vi "Anal tdms each save.vi"(5 "B Table":string[][](table), 6 "R Table":string[][](table), 7 "S Table":string[][](table), 8 "error in":errorcluster, 10 "Table Tag C":T1, 11 "TDMSファイル in":refnum<k34>) -> (0 "error out":errorcluster, 3 "TDMSファイル out":refnum<k34>)   [LabVIEW 2018]
panel:
  out "B Table Tag":string[](array[string])=["S # [n]", "S Peak Position [s]", "Signal [pA]", "Region BL [pA]", "Region STD [pA]", "Threshold [pA]", "Signal S [s]", "Signal E (s)", "S TL [ms]", "S DL [s]", "Bias [V]", "RT BL [pA]", "Chip ID [a]", "Ex ID [a]", "Distance [nm]", "EP1 [mV]", "EP2  [mV]", "Read Region Point [n", "STD [select]", "RT BL [select]", "RT STD [select]", "Moving Point [n]", "U threshold [n]", "D thereshold [n]", "STD smooth [n]", "Signal Region Point [n]", "H1 [n]", "H2 [n]"]
  out "R Table Tag":string[](array[string])=["S # [n]", "S Peak Position [s]", "Signal [pA]", "Region BL [pA]", "Region STD [pA]", "Threshold [pA]", "Signal S [s]", "Signal E (s)", "S TL [ms]", "S DL [s]", "Bias [V]", "RT BL [pA]", "Chip ID [a]", "Ex ID [a]", "Distance [nm]", "EP1 [mV]", "EP2  [mV]", "Read Region Point [n", "STD [select]", "RT BL [select]", "RT STD [select]", "Moving Point [n]", "U threshold [n]", "D thereshold [n]", "STD smooth [n]", "Signal Region Point [n]", "H1 [n]", "H2 [n]"]
  out "S Table Tag":string[](array[string])=["S # [n]", "S Peak Position [s]", "Signal [pA]", "Region BL [pA]", "Region STD [pA]", "Threshold [pA]", "Signal S [s]", "Signal E (s)", "S TL [ms]", "S DL [s]", "Bias [V]", "RT BL [pA]", "Chip ID [a]", "Ex ID [a]", "Distance [nm]", "EP1 [mV]", "EP2  [mV]", "Read Region Point [n", "STD [select]", "RT BL [select]", "RT STD [select]", "Moving Point [n]", "U threshold [n]", "D thereshold [n]", "STD smooth [n]", "Signal Region Point [n]", "H1 [n]", "H2 [n]"]
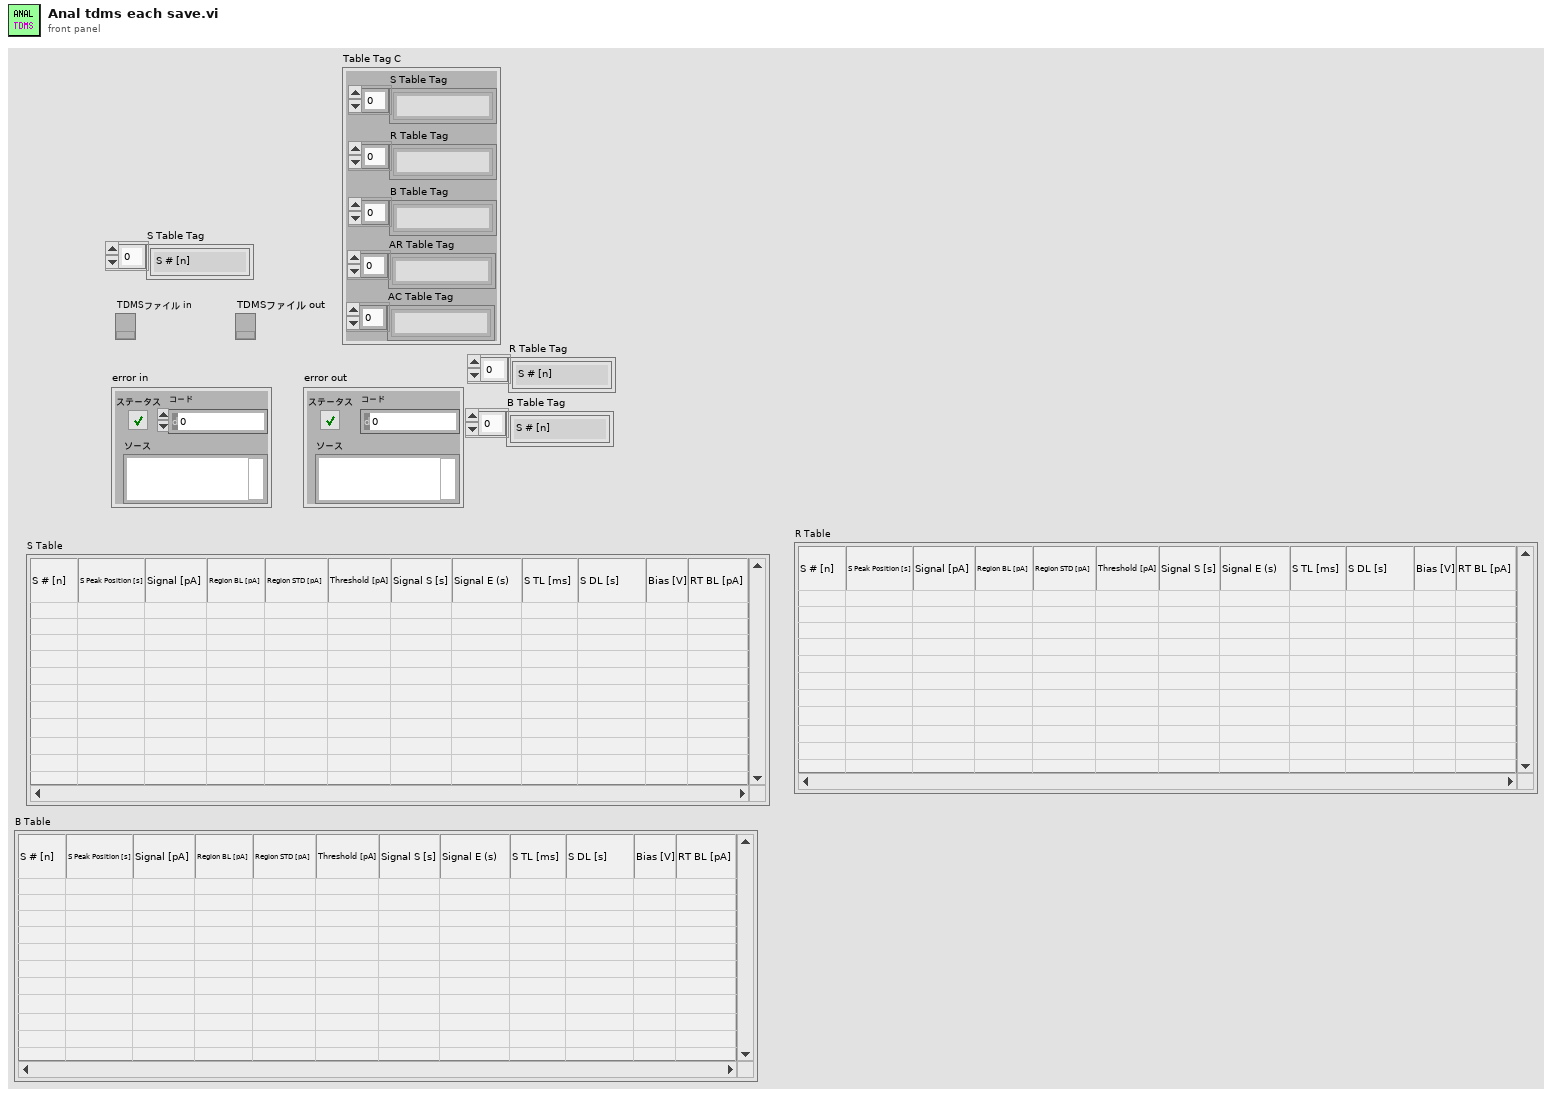
[diagram p1: front panel]
types:
  T1 = cluster{"S Table Tag":string[], "R Table Tag":string[], "B Table Tag":string[], "AR Table Tag":string[], "AC Table Tag":string[]}
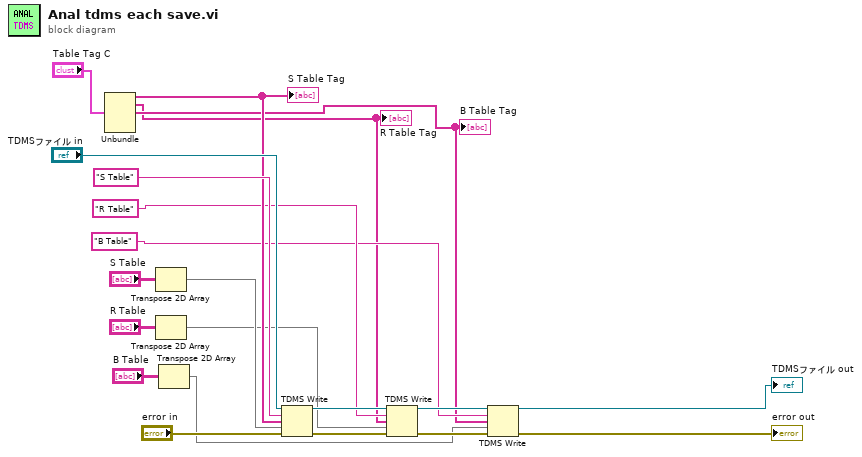
[diagram p0: block diagram]
diagram:
  n1 = Unbundle("Table Tag C") -> ("S Table Tag"=w9:string[], "R Table Tag"=w2:string[], "B Table Tag"=w3:string[])  [unwired: 2 out]
  "S Table Tag" <- w9
  "R Table Tag" <- w2
  "B Table Tag" <- w3
  n2 = Transpose 2D Array(2D array="S Table") -> (transposed array=w20:string[][])
  n3 = Transpose 2D Array(2D array="R Table") -> (transposed array=w1:string[][])
  n4 = Transpose 2D Array(2D array="B Table") -> (transposed array=w4:string[][])
  n5 = TDMS Write(0:"TDMSファイル in", 5:"S Table" ("Group name"), 7:w9, 9:w20, 11:"error in") -> (4:w15:refnum<k34>, 15:w12:errorcluster)  [unwired: 1 in, 2 out]
  n6 = TDMS Write(0:w15, 5:"R Table" ("Group name"), 7:w2, 9:w1, 11:w12) -> (4:w14:refnum<k34>, 15:w11:errorcluster)  [unwired: 1 in, 2 out]
  n7 = TDMS Write(0:w14, 5:"B Table" ("Group name"), 7:w3, 9:w4, 11:w11) -> (4:→"TDMSファイル out":refnum<k34>, 15:→"error out":errorcluster)  [unwired: 1 in, 2 out]
